vi "Destroy Request Events.vi"(8 "error in":errorcluster) -> (0 "error out":errorcluster)   [LabVIEW 2026, in "testCoordinator.lvlib"]
doc: "Destroy the requests user events, even if there is an incoming error.\n\n<b>NOTE</b>: The contents of this VI are automatically generated and modified by the <b>Tools > DQMH Consortium > DQMH</b> utilities. Consider using those utilities instead of making your own modifications to this VI.\n_____\nBased on DQMH Dev Tools: Project Template 7.1.2.1547."
uses:
  testCoordinator.lvlib
panel:
  # "NOTE: The contents of this VI are automatically generated and modified by the Tools > DQMH Consortium > DQMH utilities. Consider using those utilities instead of making your own modifications to this VI."
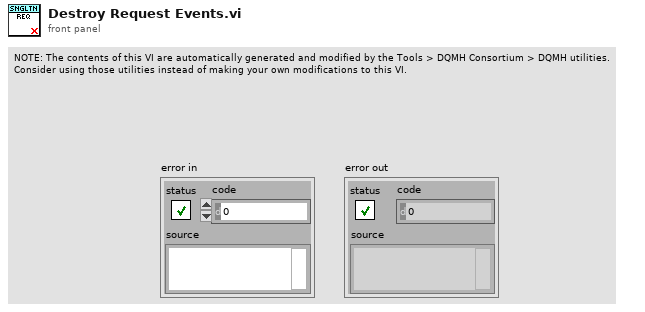
[diagram p1: front panel]
types:
  T1 = typedef "testCoordinator.lvlib/Request Events--cluster.ctl" = cluster{"Stop Module":refnum<user-event>, "Do Something":refnum<user-event>, "Do Something Else":refnum<user-event>, "Do Something Else and Wait for Reply":refnum<user-event>, "Show Panel":refnum<user-event>, "Hide Panel":refnum<user-event>, "Get Module Execution Status":refnum<user-event>, "Show Diagram":refnum<user-event>, "Set Manual Tests Folder Location":refnum<user-event>, "Private.Load Test Procedure":refnum<user-event>, "Begin Test Execution":refnum<user-event>, "Private.Process Test Procedure Metadata":refnum<user-event>, "Private.Instruction Completed":refnum<user-event>, "Private.Process First Instruction":refnum<user-event>, "Private.Load Next Test Case":refnum<user-event>, "Private.Execute Launcher":refnum<user-event>}
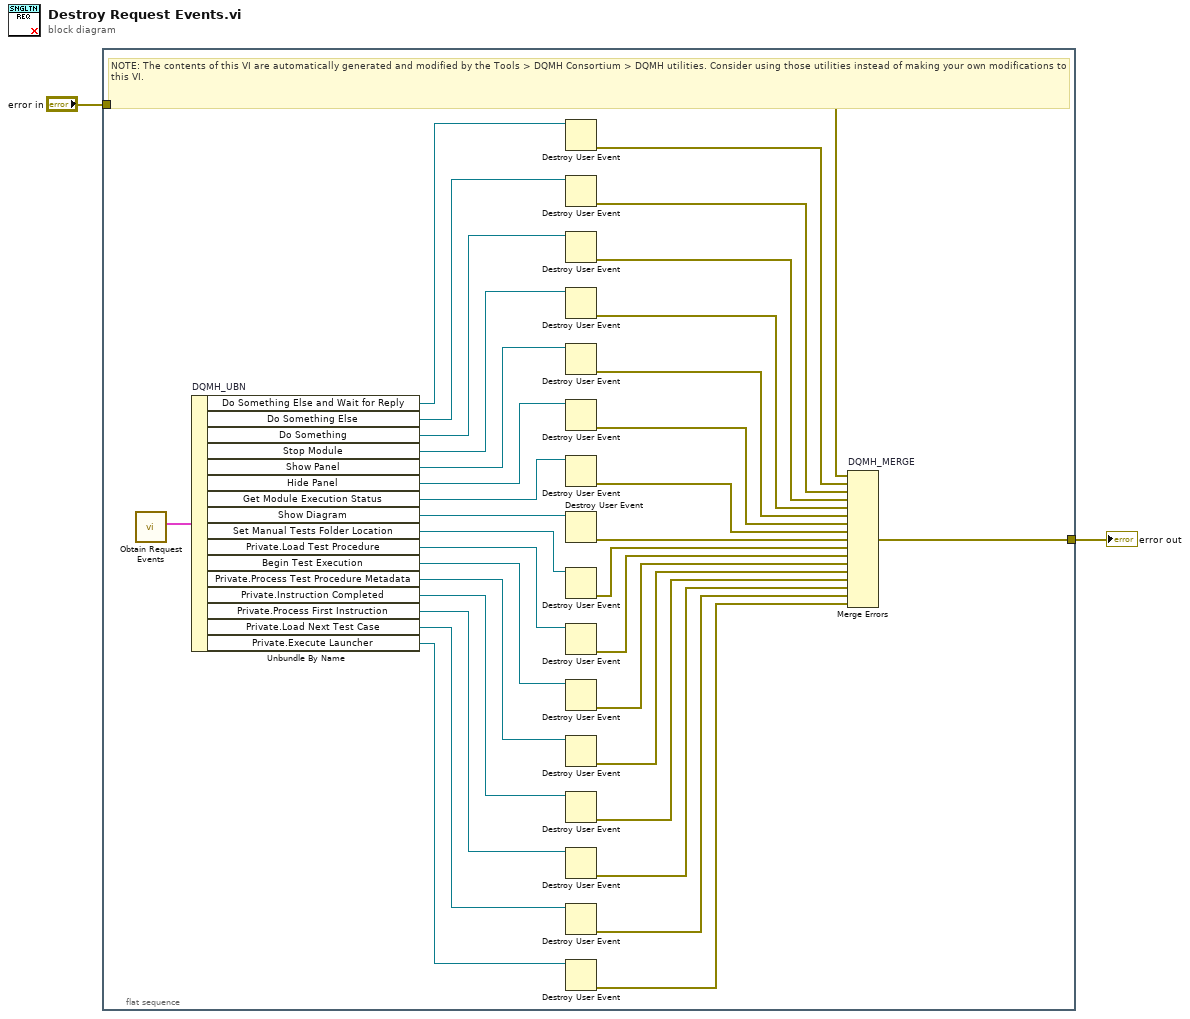
[diagram p0: block diagram]
diagram:
  n1 = flat-sequence {
    tunnel: [w36] -> w2
    tunnel: "error in" -> [w23]
    frame #0 {
      # "NOTE: The contents of this VI are automatically generated and modified by the Tools > DQMH Consortium > DQMH utilities. Consider using those utilities instead of making your own modifications to this VI."
      n2 = call "Obtain Request Events.vi"() -> ("testCoordinator Request Events"=w35:T1)  [unwired: 10 in, 1 out]
      n3 = Unbundle By Name "DQMH_UBN"(w35) -> ("Do Something Else and Wait for Reply"=w25:refnum<user-event>, "Do Something Else"=w31:refnum<user-event>, "Do Something"=w33:refnum<user-event>, "Stop Module"=w34:refnum<user-event>, "Show Panel"=w27:refnum<user-event>, "Hide Panel"=w26:refnum<user-event>, "Get Module Execution Status"=w21:refnum<user-event>, "Show Diagram"=w19:refnum<user-event>, "Set Manual Tests Folder Location"=w17:refnum<user-event>, "Private.Load Test Procedure"=w15:refnum<user-event>, "Begin Test Execution"=w13:refnum<user-event>, "Private.Process Test Procedure Metadata"=w11:refnum<user-event>, "Private.Instruction Completed"=w9:refnum<user-event>, "Private.Process First Instruction"=w7:refnum<user-event>, "Private.Load Next Test Case"=w5:refnum<user-event>, "Private.Execute Launcher"=w3:refnum<user-event>)
      n4 = Destroy User Event(user event=w25) -> (error out=w24:errorcluster)  [unwired: 1 in]
      n5 = Destroy User Event(user event=w31) -> (error out=w30:errorcluster)  [unwired: 1 in]
      n6 = Destroy User Event(user event=w33) -> (error out=w32:errorcluster)  [unwired: 1 in]
      n7 = Destroy User Event(user event=w34) -> (error out=w37:errorcluster)  [unwired: 1 in]
      n8 = Destroy User Event(user event=w27) -> (error out=w29:errorcluster)  [unwired: 1 in]
      n9 = Destroy User Event(user event=w26) -> (error out=w28:errorcluster)  [unwired: 1 in]
      n10 = Destroy User Event(user event=w21) -> (error out=w22:errorcluster)  [unwired: 1 in]
      n11 = Destroy User Event(user event=w19) -> (error out=w20:errorcluster)  [unwired: 1 in]
      n12 = Destroy User Event(user event=w17) -> (error out=w18:errorcluster)  [unwired: 1 in]
      n13 = Destroy User Event(user event=w15) -> (error out=w16:errorcluster)  [unwired: 1 in]
      n14 = Destroy User Event(user event=w13) -> (error out=w14:errorcluster)  [unwired: 1 in]
      n15 = Destroy User Event(user event=w11) -> (error out=w12:errorcluster)  [unwired: 1 in]
      n16 = Destroy User Event(user event=w9) -> (error out=w10:errorcluster)  [unwired: 1 in]
      n17 = Destroy User Event(user event=w7) -> (error out=w8:errorcluster)  [unwired: 1 in]
      n18 = Destroy User Event(user event=w5) -> (error out=w6:errorcluster)  [unwired: 1 in]
      n19 = Destroy User Event(user event=w3) -> (error out=w4:errorcluster)  [unwired: 1 in]
      n20 = Merge Errors "DQMH_MERGE"(w23, w24, w30, w32, w37, w29, w28, w22, w20, w18, w16, w14, w12, w10, w8, w6, w4) -> (w36:errorcluster)
    }
  }
  "error out" <- w2
